vi "SubTask3.vi"   [LabVIEW 2016]
uses:
  <vilib>/NXT/Block Support/NXT_OutputPort.ctl
  <vilib>/NXT/Block Support/NXT_InputPort.ctl
  <vilib>/NXT/Dual Mode Library/Sensors/EV3_Color_Color.vi
  <vilib>/NXT/Dual Mode Library/Sensors/EV3_Ultrasonic_CM.vi
  <vilib>/NXT/NXTIO Xnodes/NXTIONodeSubVIs/NXTMoveMotors.vi
  <vilib>/NXT/NXTIO Xnodes/NXTIONodeSubVIs/NXTStopMotors.vi
  <vilib>/NXT/Dual Mode Library/Motors/Rotation.vi
  <vilib>/NXT/Dual Mode Library/Display/drawText_Center.vi
  <vilib>/NXT/Dual Mode Library/Waits/Wait_Num.vi
  <vilib>/NXT/Dual Mode Library/Display/drawNumber.vi
  <vilib>/NXT/Dual Mode Library/Motors/ResetMotor.vi
  <vilib>/NXT/NXTIO Xnodes/AddressXNode/NXTIOAddress.xnode
  PMR_081.lvrbt
  <vilib>/NXT/Subs/LVHSConnector.ctl
  <vilib>/NXT/NXTIO Xnodes/NXTIOXNode/NXTIO.xnode
  <vilib>/NXT/LegoClasses/BrickReference/BrickReference.lvclass
types:
  T1 = typedef "NXT_OutputPort.ctl" = u8
  T2 = typedef "NXT_InputPort.ctl" = u32
  T3 = typedef "ColorSensorColors.ctl" = enum16{"No Color", "Black", "Blue", "Green", "Yellow", "Red", "White", "Brown"}
  T4 = typedef "LVHSConnector.ctl" = refnum<class "BrickReference.lvclass">
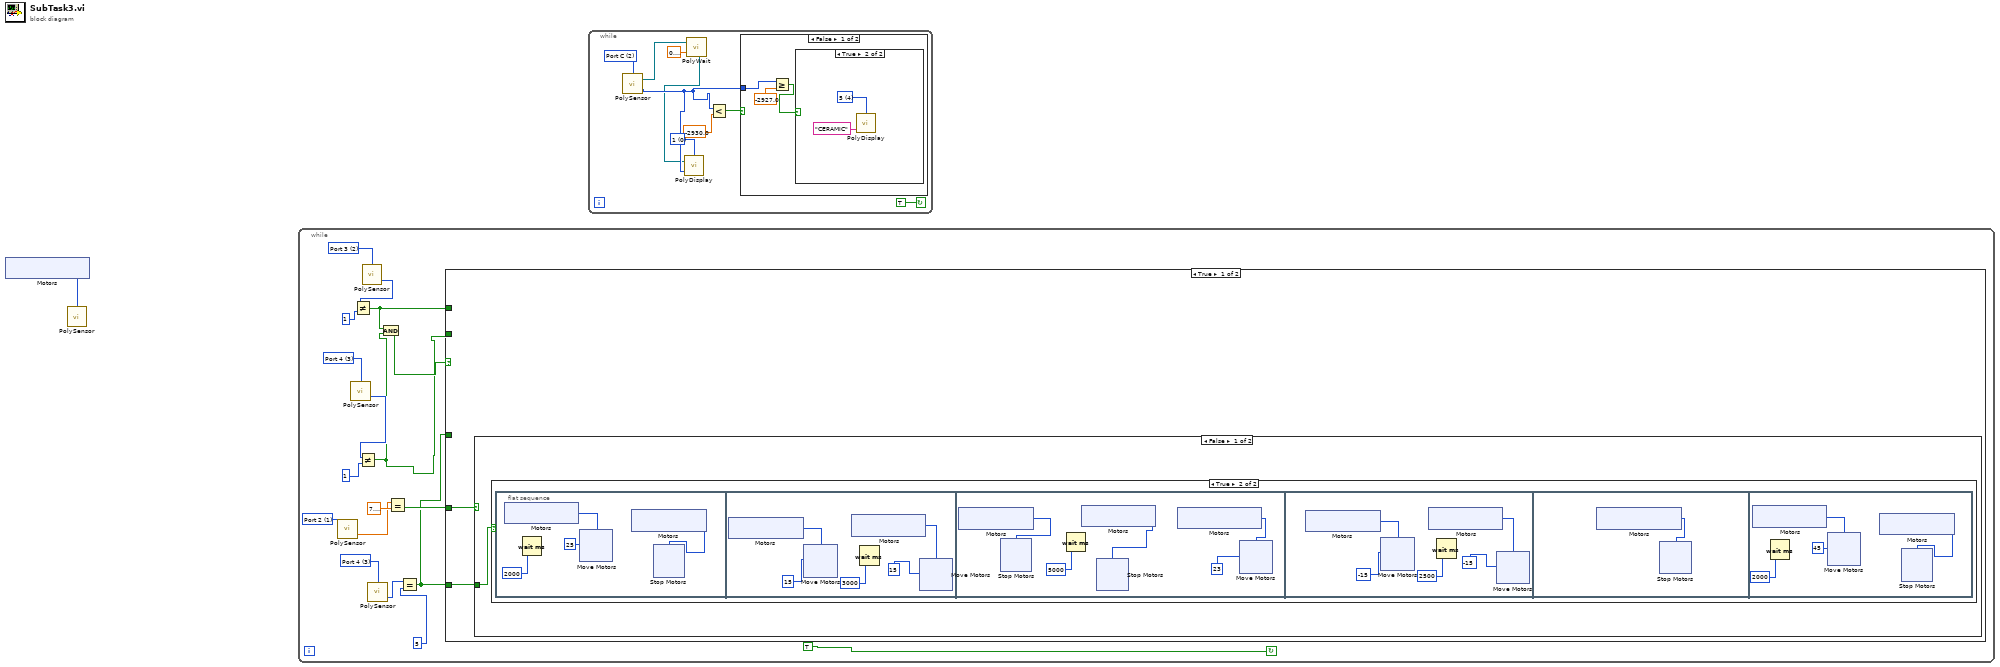
[diagram p0: block diagram]
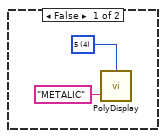
[diagram p2: hidden frame]
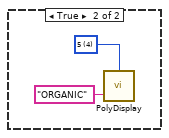
[diagram p3: hidden frame]
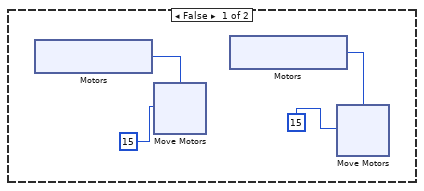
[diagram p4: hidden frame]
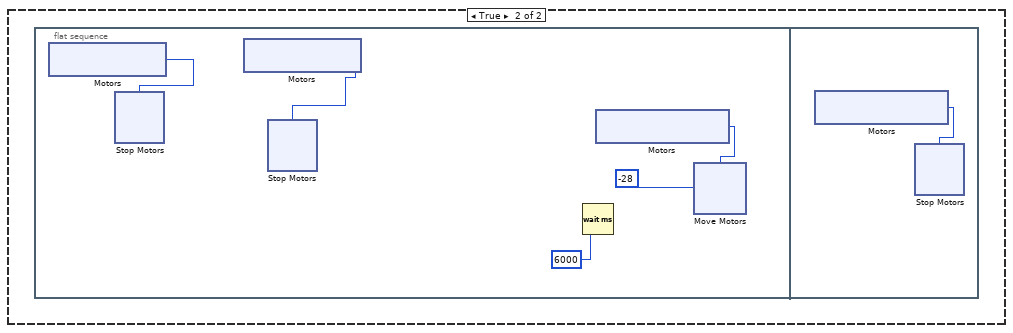
[diagram p5: hidden frame]
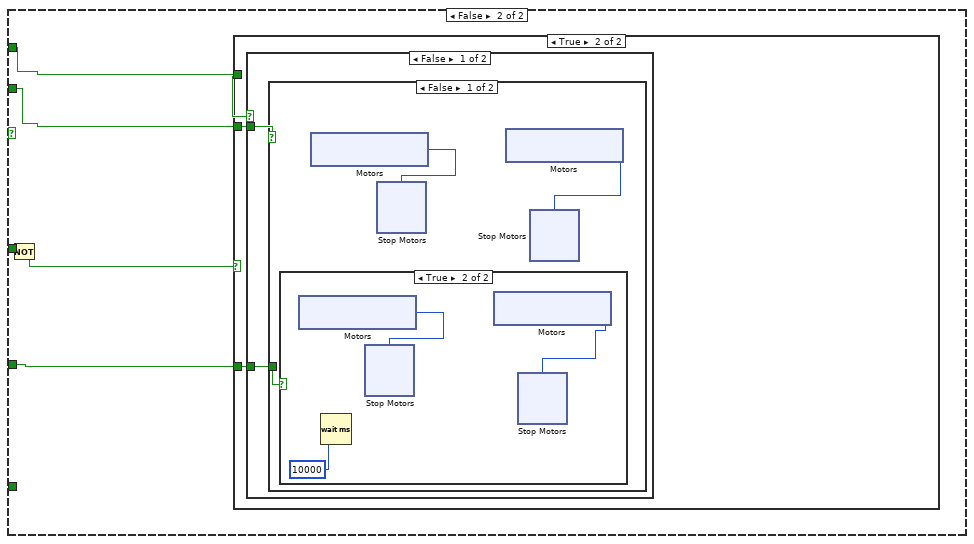
[diagram p6: hidden frame]
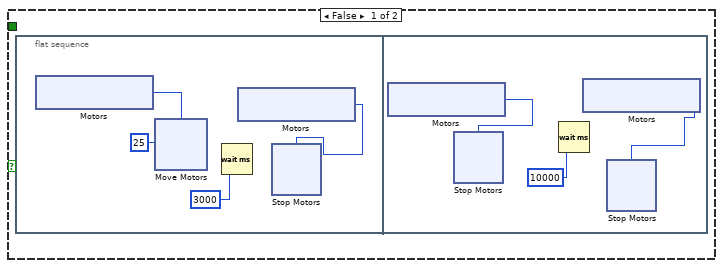
[diagram p7: hidden frame]
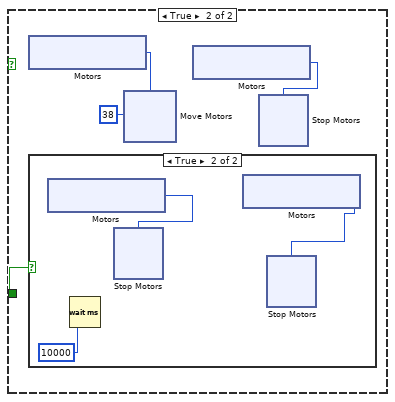
[diagram p9: hidden frame]
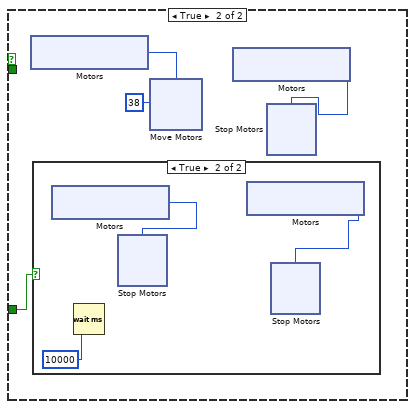
[diagram p11: hidden frame]
diagram:
  n1 = xnode "Motors"() -> ("Motor"=w1:T1)
  n2 = call-poly <vilib>:"PolySensor.vi"("Port (All Ports)"=w1) -> ()  [unwired: 3 in, 1 out]
  n3 = while {
    stop <- TRUE continue-if-true
    w5 = T2 3 items=["Port 1", "Port 2", "Port 3", "Port 4"] ("Port (Port 1)")
    w8 = T2 1 items=["Port 1", "Port 2", "Port 3", "Port 4"] ("Port (Port 4)")
    w18 = T2 3 items=["Port 1", "Port 2", "Port 3", "Port 4"] ("Port (Port 1)")
    w19 = T2 2 items=["Port 1", "Port 2", "Port 3", "Port 4"] ("Port (Port 1)")
    n4 = call-poly <vilib>:"PolySensor.vi"("Port (Port 1)"=w8) -> ("Centimeters"=w7:sgl)  [unwired: 2 in, 1 out]
    n5 = call-poly <vilib>:"PolySensor.vi"("Port (Port 1)"=w18) -> ("Detected Color"=w14:T3)  [unwired: 2 in, 1 out]
    n6 = Not Equal?(x=w14, y=1) -> (x != y?=w10:bool)
    n7 = call-poly <vilib>:"PolySensor.vi"("Port (Port 1)"=w19) -> ("Detected Color"=w16:T3)  [unwired: 2 in, 1 out]
    n8 = Not Equal?(x=w16, y=1) -> (x != y?=w12:bool)
    n9 = call-poly <vilib>:"PolySensor.vi"("Port (Port 1)"=w5) -> ("Detected Color"=w4:T3)  [unwired: 2 in, 1 out]
    n10 = And(x=w12, y=w10) -> (x .and. y?=w11:bool)
    n11 = Equal?(x=w7, y=sgl 7.2) -> (x = y?=w6:bool)
    n12 = Equal?(x=w4, y=5) -> (x = y?=w2:bool)
    n13 = case shown="True" w11 {
      tunnel: w12 -> [_ w189]
      tunnel: w10 -> [_ w188]
      tunnel: w6 -> [w21 w187]
      tunnel: w2 -> [w20 _]
      tunnel: w2 -> [_ w186]
      frame True {
        n14 = case shown="False" w21 {
          tunnel: w20 -> [w22 _]
          frame False {
            n15 = case shown="True" w22 {
              frame False {
                n16 = xnode "Motors"() -> ("Motor"=w25:T1)
                n17 = xnode "Move Motors"("Power/Speed 1"=i8 15, "Motors"=w25) -> ()  [unwired: 1 in, 1 out]
                n18 = xnode "Motors"() -> ("Motor"=w26:T1)
                n19 = xnode "Move Motors"("Power/Speed 1"=i8 15, "Motors"=w26) -> ()  [unwired: 1 in, 1 out]
              }
              frame True {
                n20 = flat-sequence {
                  frame #0 {
                    n21 = xnode "Motors"() -> ("Motor"=w45:T1)
                    n22 = Wait (ms)(milliseconds to wait=2000) -> ()  [unwired: 1 out]
                    n23 = xnode "Move Motors"("Power/Speed 1"=i8 25, "Motors"=w45) -> ()  [unwired: 1 in, 1 out]
                    n24 = xnode "Motors"() -> ("Motor"=w44:T1)
                    n25 = xnode "Stop Motors"("Motors"=w44) -> ()  [unwired: 1 in, 1 out]
                  }
                  frame #1 {
                    n26 = xnode "Motors"() -> ("Motor"=w64:T1)
                    n27 = xnode "Move Motors"("Power/Speed 1"=i8 15, "Motors"=w64) -> ()  [unwired: 1 in, 1 out]
                    n28 = xnode "Motors"() -> ("Motor"=w65:T1)
                    n29 = Wait (ms)(milliseconds to wait=3000) -> ()  [unwired: 1 out]
                    n30 = xnode "Move Motors"("Power/Speed 1"=i8 15, "Motors"=w65) -> ()  [unwired: 1 in, 1 out]
                  }
                  frame #2 {
                    n31 = xnode "Motors"() -> ("Motor"=w85:T1)
                    n32 = xnode "Stop Motors"("Motors"=w85) -> ()  [unwired: 1 in, 1 out]
                    n33 = Wait (ms)(milliseconds to wait=5000) -> ()  [unwired: 1 out]
                    n34 = xnode "Motors"() -> ("Motor"=w84:T1)
                    n35 = xnode "Stop Motors"("Motors"=w84) -> ()  [unwired: 1 in, 1 out]
                    n36 = xnode "Motors"() -> ("Motor"=w82:T1)
                    n37 = xnode "Move Motors"("Power/Speed 1"=23, "Motors"=w82) -> ()  [unwired: 1 in, 1 out]
                  }
                  frame #3 {
                    n38 = xnode "Motors"() -> ("Motor"=w110:T1)
                    n39 = xnode "Move Motors"("Power/Speed 1"=i8 -15, "Motors"=w110) -> ()  [unwired: 1 in, 1 out]
                    n40 = xnode "Motors"() -> ("Motor"=w111:T1)
                    n41 = Wait (ms)(milliseconds to wait=2500) -> ()  [unwired: 1 out]
                    n42 = xnode "Move Motors"("Power/Speed 1"=i8 -15, "Motors"=w111) -> ()  [unwired: 1 in, 1 out]
                  }
                  frame #4 {
                    n43 = xnode "Motors"() -> ("Motor"=w128:T1)
                    n44 = xnode "Stop Motors"("Motors"=w128) -> ()  [unwired: 1 in, 1 out]
                  }
                  frame #5 {
                    n45 = xnode "Motors"() -> ("Motor"=w136:T1)
                    n46 = Wait (ms)(milliseconds to wait=2000) -> ()  [unwired: 1 out]
                    n47 = xnode "Move Motors"("Power/Speed 1"=i8 45, "Motors"=w136) -> ()  [unwired: 1 in, 1 out]
                    n48 = xnode "Motors"() -> ("Motor"=w137:T1)
                    n49 = xnode "Stop Motors"("Motors"=w137) -> ()  [unwired: 1 in, 1 out]
                  }
                }
              }
            }
          }
          frame True {
            n50 = flat-sequence {
              frame #0 {
                n51 = xnode "Motors"() -> ("Motor"=w157:T1)
                n52 = xnode "Stop Motors"("Motors"=w157) -> ()  [unwired: 1 in, 1 out]
                n53 = xnode "Motors"() -> ("Motor"=w156:T1)
                n54 = xnode "Stop Motors"("Motors"=w156) -> ()  [unwired: 1 in, 1 out]
                n55 = Wait (ms)(milliseconds to wait=6000) -> ()  [unwired: 1 out]
                n56 = xnode "Motors"() -> ("Motor"=w153:T1)
                n57 = xnode "Move Motors"("Power/Speed 1"=-28, "Motors"=w153) -> ()  [unwired: 1 in, 1 out]
              }
              frame #1 {
                n58 = xnode "Motors"() -> ("Motor"=w178:T1)
                n59 = xnode "Stop Motors"("Motors"=w178) -> ()  [unwired: 1 in, 1 out]
              }
            }
          }
        }
      }
      frame False {
        n60 = Not(x=w186) -> (.not. x?=w185:bool)
        n61 = case shown="True" w185 {
          tunnel: w189 -> [_ w225]
          tunnel: w188 -> [_ w224]
          tunnel: w187 -> [_ w223]
          frame False {
            n62 = flat-sequence {
              frame #0 {
                n63 = xnode "Motors"() -> ("Motor"=w192:T1)
                n64 = xnode "Move Motors"("Power/Speed 1"=i8 25, "Motors"=w192) -> ()  [unwired: 1 in, 1 out]
                n65 = Wait (ms)(milliseconds to wait=3000) -> ()  [unwired: 1 out]
                n66 = xnode "Motors"() -> ("Motor"=w191:T1)
                n67 = xnode "Stop Motors"("Motors"=w191) -> ()  [unwired: 1 in, 1 out]
              }
              frame #1 {
                n68 = xnode "Motors"() -> ("Motor"=w209:T1)
                n69 = xnode "Stop Motors"("Motors"=w209) -> ()  [unwired: 1 in, 1 out]
                n70 = Wait (ms)(milliseconds to wait=10000) -> ()  [unwired: 1 out]
                n71 = xnode "Motors"() -> ("Motor"=w208:T1)
                n72 = xnode "Stop Motors"("Motors"=w208) -> ()  [unwired: 1 in, 1 out]
              }
            }
          }
          frame True {
            n73 = case shown="False" w225 {
              tunnel: w224 -> [w227 _]
              tunnel: w223 -> [w226 w291]
              frame False {
                n74 = case shown="False" w227 {
                  tunnel: w226 -> [w228 w258]
                  frame False {
                    n75 = case shown="True" w228 {
                      frame False {
                      }
                      frame True {
                        n76 = xnode "Motors"() -> ("Motor"=w232:T1)
                        n77 = Wait (ms)(milliseconds to wait=10000) -> ()  [unwired: 1 out]
                        n78 = xnode "Stop Motors"("Motors"=w232) -> ()  [unwired: 1 in, 1 out]
                        n79 = xnode "Motors"() -> ("Motor"=w231:T1)
                        n80 = xnode "Stop Motors"("Motors"=w231) -> ()  [unwired: 1 in, 1 out]
                      }
                    }
                    n81 = xnode "Motors"() -> ("Motor"=w229:T1)
                    n82 = xnode "Stop Motors"("Motors"=w229) -> ()  [unwired: 1 in, 1 out]
                    n83 = xnode "Motors"() -> ("Motor"=w230:T1)
                    n84 = xnode "Stop Motors"("Motors"=w230) -> ()  [unwired: 1 in, 1 out]
                  }
                  frame True {
                    n85 = xnode "Motors"() -> ("Motor"=w260:T1)
                    n86 = case shown="True" w258 {
                      frame False {
                      }
                      frame True {
                        n87 = xnode "Motors"() -> ("Motor"=w263:T1)
                        n88 = Wait (ms)(milliseconds to wait=10000) -> ()  [unwired: 1 out]
                        n89 = xnode "Stop Motors"("Motors"=w263) -> ()  [unwired: 1 in, 1 out]
                        n90 = xnode "Motors"() -> ("Motor"=w262:T1)
                        n91 = xnode "Stop Motors"("Motors"=w262) -> ()  [unwired: 1 in, 1 out]
                      }
                    }
                    n92 = xnode "Move Motors"("Power/Speed 1"=i8 38, "Motors"=w260) -> ()  [unwired: 1 in, 1 out]
                    n93 = xnode "Motors"() -> ("Motor"=w261:T1)
                    n94 = xnode "Stop Motors"("Motors"=w261) -> ()  [unwired: 1 in, 1 out]
                  }
                }
              }
              frame True {
                n95 = xnode "Motors"() -> ("Motor"=w293:T1)
                n96 = case shown="True" w291 {
                  frame False {
                  }
                  frame True {
                    n97 = xnode "Motors"() -> ("Motor"=w301:T1)
                    n98 = Wait (ms)(milliseconds to wait=10000) -> ()  [unwired: 1 out]
                    n99 = xnode "Stop Motors"("Motors"=w301) -> ()  [unwired: 1 in, 1 out]
                    n100 = xnode "Motors"() -> ("Motor"=w300:T1)
                    n101 = xnode "Stop Motors"("Motors"=w300) -> ()  [unwired: 1 in, 1 out]
                  }
                }
                n102 = xnode "Move Motors"("Power/Speed 1"=i8 38, "Motors"=w293) -> ()  [unwired: 1 in, 1 out]
                n103 = xnode "Motors"() -> ("Motor"=w292:T1)
                n104 = xnode "Stop Motors"("Motors"=w292) -> ()  [unwired: 1 in, 1 out]
              }
            }
          }
        }
      }
    }
  }
  n105 = while {
    stop <- TRUE continue-if-true
    w328 = i16 0 items=["1", "2", "3", "4", "5", "6", "7", "8", "9", "10", "11", "12"] ("Line")
    w329 = T1 2 items=["Port A", "Port B", "Port C", "Port D"] ("Port (Port A)")
    n106 = call-poly <vilib>:"PolySensor.vi"("Port (Port A)"=w329) -> ("Angle of Rotation"=w327:i32, "NXT/EV3"=w326:T4)  [unwired: 2 in]
    n107 = call-poly <vilib>:"PolyWait.vi"("Time (1 sec)"=sgl 0.3, "NXT/EV3"=w326) -> ("NXT/EV3"=w325:T4)  [unwired: 2 in]
    n108 = call-poly <vilib>:"PolyDisplay.vi"("number"=w327, "NXT/EV3"=w325, "Line"=w328) -> ()  [unwired: 1 in, 1 out]
    n109 = Less?(x=w327, y=sgl -2930.0) -> (x < y?=w331:bool)
    n110 = case shown="False" w331 {
      tunnel: w327 -> [w334 _]
      frame False {
        n111 = Greater Or Equal?(x=w334, y=sgl -2927.0) -> (x >= y?=w333:bool)
        n112 = case shown="True" w333 {
          frame False {
            w336 = i16 4 items=["1", "2", "3", "4", "5", "6", "7", "8", "9", "10", "11", "12"] ("Line")
            n113 = call-poly <vilib>:"PolyDisplay.vi"("Text"="METALIC", "Line"=w336) -> ()  [unwired: 2 in, 1 out]
          }
          frame True {
            w338 = i16 4 items=["1", "2", "3", "4", "5", "6", "7", "8", "9", "10", "11", "12"] ("Line")
            n114 = call-poly <vilib>:"PolyDisplay.vi"("Text"="CERAMIC", "Line"=w338) -> ()  [unwired: 2 in, 1 out]
          }
        }
      }
      frame True {
        w340 = i16 4 items=["1", "2", "3", "4", "5", "6", "7", "8", "9", "10", "11", "12"] ("Line")
        n115 = call-poly <vilib>:"PolyDisplay.vi"("Text"="ORGANIC", "Line"=w340) -> ()  [unwired: 2 in, 1 out]
      }
    }
  }
